vi "[ce] Differentiation.vi"(5 "h":dbl=1e-08 format="%.2e", 6 "parameters":cluster{"name":string, "value":dbl}[](array[cluster]) {"value" format="%.2f"}, 7 "# points":u32=100, 8 "error in":errorcluster, 9 "formula info":cluster{"formula":string, "x-variable":string}={"formula"="", "x-variable"="x"}, 10 "end":dbl=1.0 format="%.2f", 11 "start":dbl format="%.2f") -> (0 "error out":errorcluster, 1 "Derivative of Y":dbl[](array[numeric]) format="%.2f", 2 "Y Values":dbl[](array[numeric]) format="%.2f", 3 "X Values":dbl[](array[numeric]) format="%.2f", 4 "ticks":u32)   [LabVIEW 2021]
doc: "Calculates both function values and the values of the derivative of 1D function defined by a formula. \nThe VI allows specifying additional parameters and evaluating them in formula.\n\n::: CalcExpress Toolkit :::\nCopyright (c) 2000-2026 Konstantin Shifershteyn. All rights reserved."
panel:
  # "Example 1:\n---------------\nformula info:\n  formula: sin(t)+cos(t)\n  x-variable: t\nparameters:  empty array\n\nExample 2:\n---------------\nformula info:\n  formula: a*sin(x)*exp(-x/b)\n  x-variable: x\nparameters: (a,1), (b,2)"
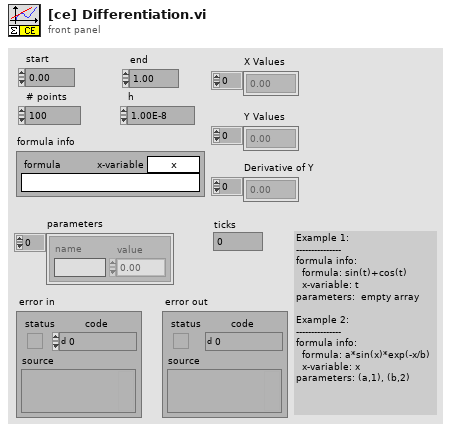
[diagram p1: front panel]
types:
  T1 = enum16{"create", "destroy", "set value", "get value"}
  T2 = typedef "VarMan Variable Context Handle.ctl" = i32
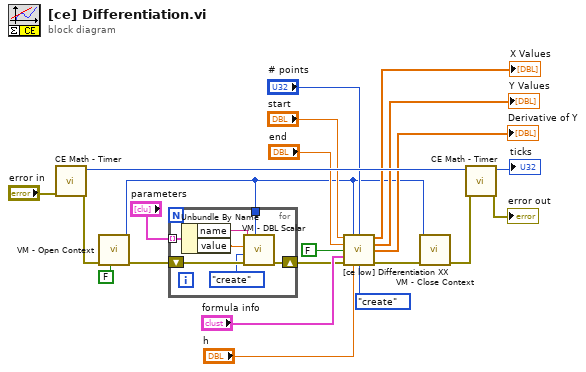
[diagram p0: block diagram]
diagram:
  n1 = call "CE Math - Timer.vi"("error in (no error)"="error in") -> ("error out"=w22:errorcluster, "ticks out"=w20:u32)  [unwired: 7 in]
  n2 = call "VM - Open Context.vi"("close loose contexts (F)"=FALSE ("close loose contexts (T)"), "error in"=w22) -> ("error out"=w5:errorcluster, "VC Handle out"=w4:T2)  [unwired: 7 in, 1 out]
  n3 = for {
    shift-right: [w26] -> w6
    shift-left: w5 -> [w27]
    tunnel: "parameters" -> [w24] mode=indexing
    tunnel: w4 -> [w23]
    n4 = Unbundle By Name(w24) -> ("name"=w28:string, "value"=w29:dbl)
    n5 = call "VM - DBL Scalar.vi"("VC Handle"=w23, "error in"=w27, "cmd"=T1."create", "value in"=w29, "name_spec"=w28) -> ("error out"=w26:errorcluster)  [unwired: 1 in, 5 out]
  }
  n6 = call "[ce low] Differentiation XX.vi"("start"="start", "VC Handle"=w4, "# points"="# points", "end"="end", "include end point"=FALSE ("w final point"), "formula info"="formula info", "error in"=w6, "h"="h", "vm cmd"=T1."create") -> ("X Values"=→"X Values":dbl[], "Y Values"=→"Y Values":dbl[], "Derivative of Y"=→"Derivative of Y":dbl[], "error out"=w21:errorcluster)  [unwired: 2 in, 1 out]
  n7 = call "VM - Close Context.vi"("error in"=w21, "VC Handle"=w4) -> ("error out"=w19:errorcluster)  [unwired: 8 in, 1 out]
  n8 = call "CE Math - Timer.vi"("error in (no error)"=w19, "ticks in"=w20) -> ("error out"=→"error out":errorcluster, "ticks out"=→"ticks":u32)  [unwired: 6 in]
